vi "Depth count VI.vi"(5 "MS_Total Con and T":cluster{dbl[], dbl[], dbl[], dbl[], i32[]}, 6 "Date":string, 7 "Total Con and T":T1, 8 "error in":errorcluster caption="エラー入力", 9 "Folder Path":string, 10 "Sample Sequence":string, 11 "Cutted Sample Sequence":string) -> (0 "error out":errorcluster caption="エラー出力")   [LabVIEW 2018]
panel:
  out "MS_B Table":string[][](table) caption="B Table"
  out "B Table":string[][](table)
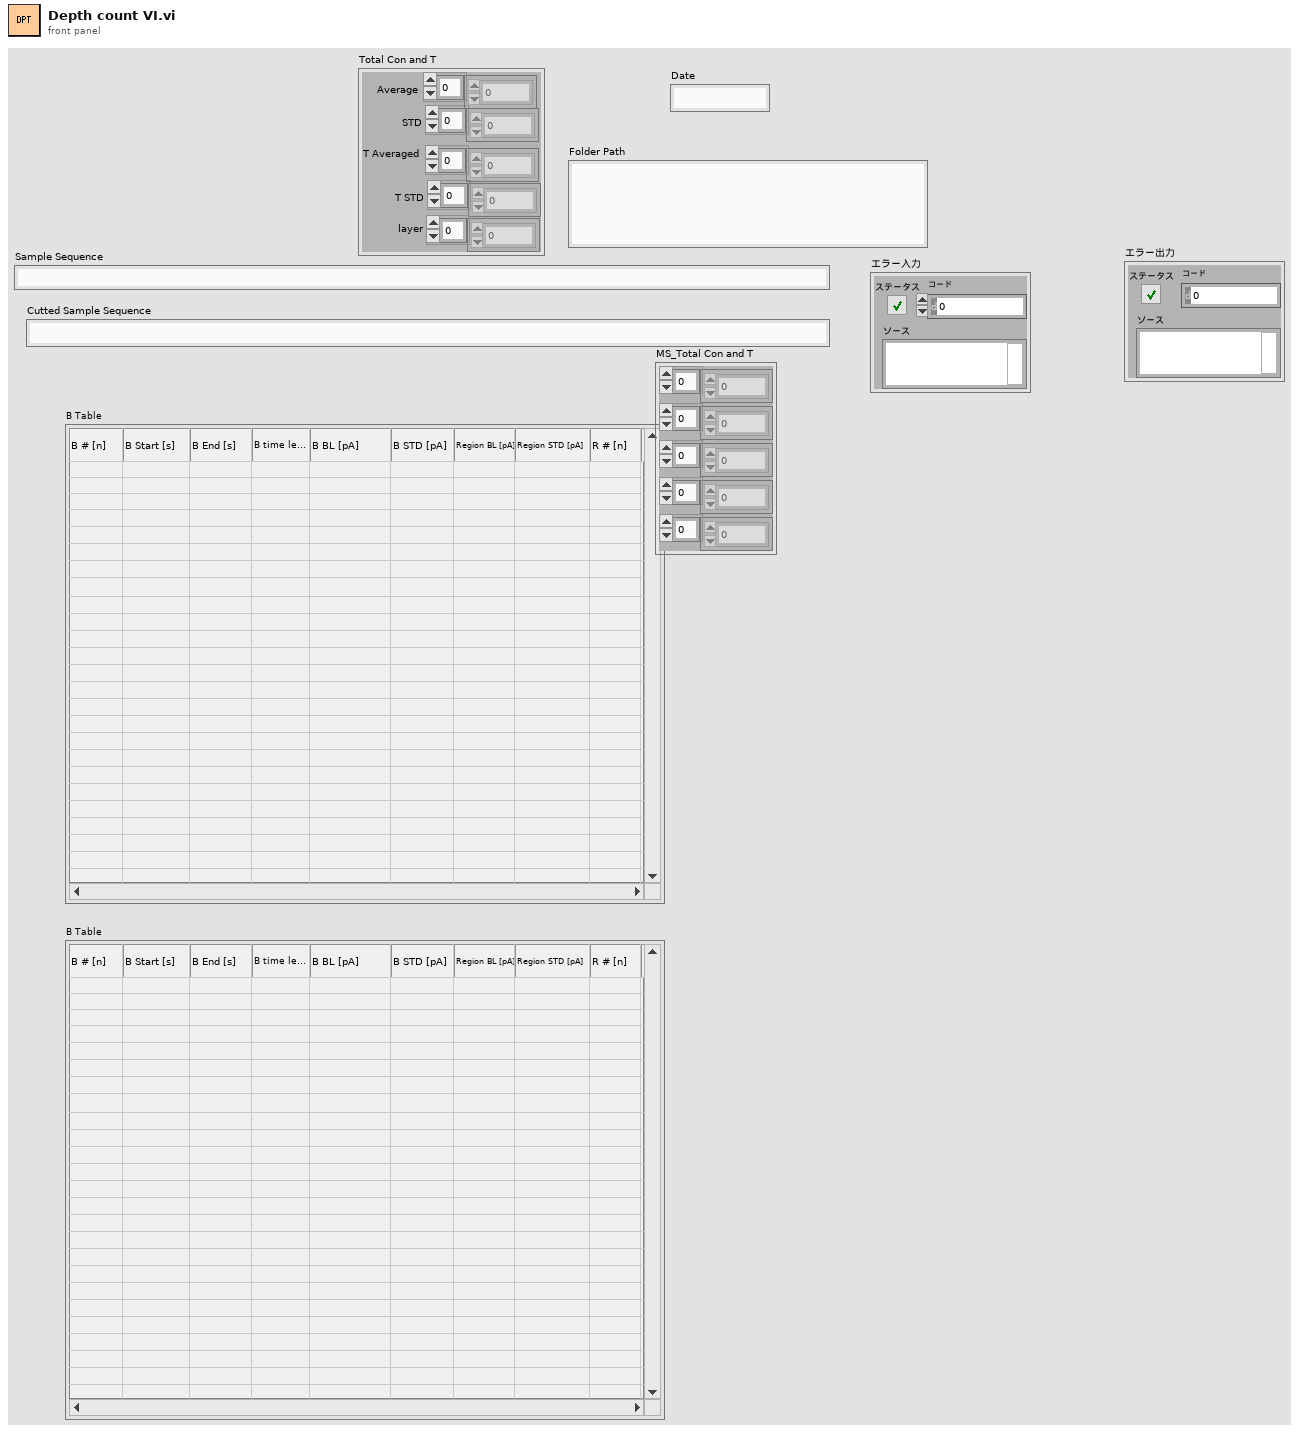
[diagram p1: front panel]
types:
  T1 = cluster{"Average":dbl[], "STD":dbl[], "T Averaged":dbl[], "T STD":dbl[], "layer":i32[]}
  T2 = enum16{"open", "replace", "create", "open or create", "replace or create", "replace or create with confirmation"}
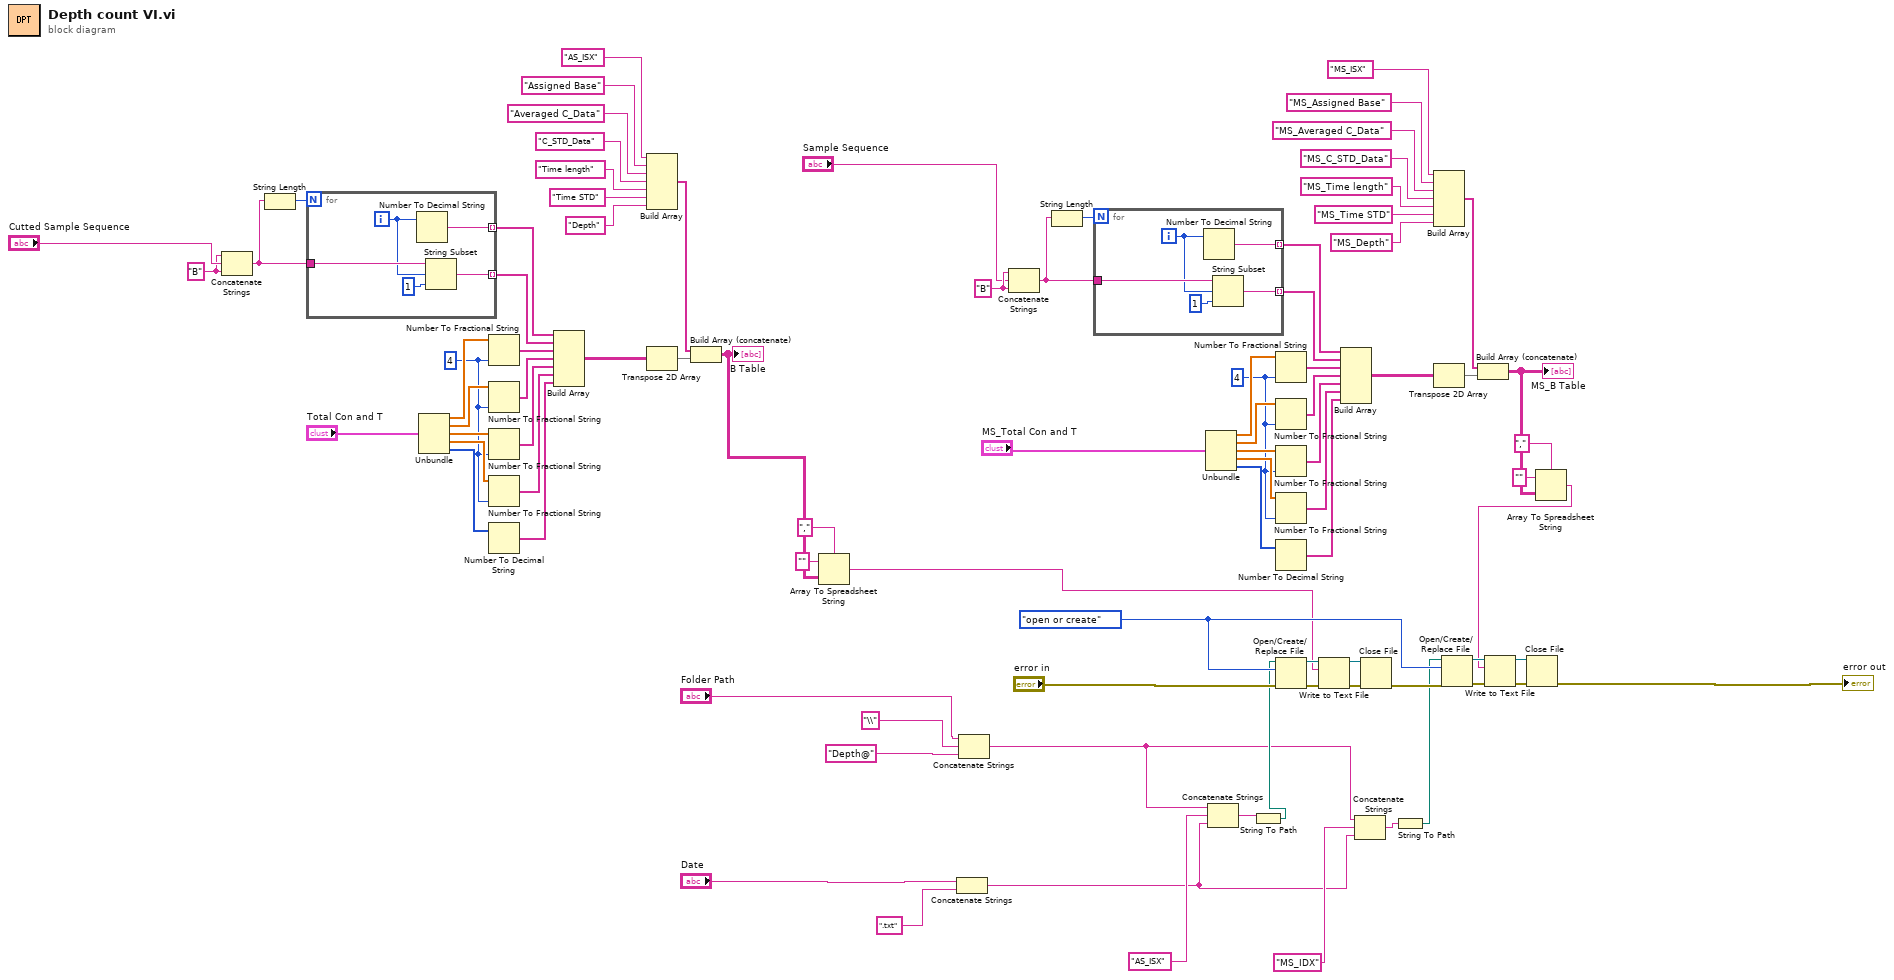
[diagram p0: block diagram]
diagram:
  w21 = T2."open or create" ("操作（0:open）")
  w49 = "B" ("string")
  w56 = i16 4 ("precision (6)")
  w75 = "B" ("string")
  w83 = i16 4 ("precision (6)")
  n1 = Concatenate Strings(w75, "Cutted Sample Sequence", w75) -> (w73:string)
  n2 = String Length(string=w73) -> (length=w74:i32)
  n3 = for {
    N: w74 -> [_]
    tunnel: w73 -> [w93]
    tunnel: [w92] -> w71 mode=indexing
    tunnel: [w90] -> w72 mode=indexing
    i -> [w91]
    n4 = Number To Decimal String(number=w91) -> (decimal integer string=w90:string)  [unwired: 1 in]
    n5 = String Subset(string=w93, offset (0)=w91, length (rest)=1 ("length (rest)")) -> (substring=w92:string)
  }
  n6 = Unbundle("Total Con and T") -> ("Average"=w88:dbl[], "STD"=w87:dbl[], "T Averaged"=w86:dbl[], "T STD"=w85:dbl[], "layer"=w84:i32[])
  n7 = Number To Fractional String(number=w88, precision (6)=w83) -> (F-format string=w82:string[])  [unwired: 2 in]
  n8 = Number To Fractional String(number=w87, precision (6)=w83) -> (F-format string=w81:string[])  [unwired: 2 in]
  n9 = Number To Fractional String(number=w86, precision (6)=w83) -> (F-format string=w80:string[])  [unwired: 2 in]
  n10 = Number To Fractional String(number=w85, precision (6)=w83) -> (F-format string=w79:string[])  [unwired: 2 in]
  n11 = Number To Decimal String(number=w84) -> (decimal integer string=w78:string[])  [unwired: 1 in]
  n12 = Build Array(w72, w71, w82, w81, w80, w79, w78) -> (w77:string[][])
  n13 = Build Array("AS_ISX" ("string"), "Assigned Base" ("string"), "Averaged C_Data" ("string"), "C_STD_Data" ("string"), "Time length" ("string"), "Time STD" ("string"), "Depth" ("string")) -> (w62:string[])
  n14 = Transpose 2D Array(2D array=w77) -> (transposed array=w63:string[][])
  n15 = Build Array (concatenate)(w62, w63) -> (w2:string[][])
  "B Table" <- w2
  n16 = Array To Spreadsheet String(delimiter (Tab)=",", array=w2, 3:"" ("format string")) -> (spreadsheet string=w1:string)
  n17 = Concatenate Strings("Date", ".txt" ("文字列")) -> (w12:string)
  n18 = Concatenate Strings("Folder Path", "\\" ("文字列"), "Depth@" ("文字列")) -> (w11:string)
  n19 = Concatenate Strings(w49, "Sample Sequence", w49) -> (w47:string)
  n20 = String Length(string=w47) -> (length=w48:i32)
  n21 = for {
    N: w48 -> [_]
    tunnel: w47 -> [w98]
    tunnel: [w97] -> w45 mode=indexing
    tunnel: [w95] -> w46 mode=indexing
    i -> [w96]
    n22 = Number To Decimal String(number=w96) -> (decimal integer string=w95:string)  [unwired: 1 in]
    n23 = String Subset(string=w98, offset (0)=w96, length (rest)=1 ("length (rest)")) -> (substring=w97:string)
  }
  n24 = Unbundle("MS_Total Con and T") -> (w61:dbl[], w60:dbl[], w59:dbl[], w58:dbl[], w57:i32[])
  n25 = Concatenate Strings(w11, "AS_ISX" ("文字列"), w12) -> (w16:string)
  n26 = String To Path(string=w16) -> (path=w15:path)
  n27 = Number To Fractional String(number=w61, precision (6)=w56) -> (F-format string=w55:string[])  [unwired: 2 in]
  n28 = Number To Fractional String(number=w60, precision (6)=w56) -> (F-format string=w54:string[])  [unwired: 2 in]
  n29 = Number To Fractional String(number=w59, precision (6)=w56) -> (F-format string=w53:string[])  [unwired: 2 in]
  n30 = Number To Fractional String(number=w58, precision (6)=w56) -> (F-format string=w52:string[])  [unwired: 2 in]
  n31 = Number To Decimal String(number=w57) -> (decimal integer string=w51:string[])  [unwired: 1 in]
  n32 = Open/Create/Replace File(file path (use dialog)=w15, error in="error in", operation (0:open)=w21) -> (refnum out=w30:refnum<file>, error out=w31:errorcluster)  [unwired: 3 in, 1 out]
  n33 = Write to Text File(file (use dialog)=w30, text=w1, error in=w31) -> (refnum out=w29:refnum<file>, error out=w28:errorcluster)  [unwired: 1 in, 1 out]
  n34 = Build Array(w46, w45, w55, w54, w53, w52, w51) -> (w50:string[][])
  n35 = Concatenate Strings(w11, "MS_IDX" ("文字列"), w12) -> (w14:string)
  n36 = Close File(refnum=w29, error in=w28) -> (error out=w22:errorcluster)  [unwired: 1 out]
  n37 = String To Path(string=w14) -> (path=w13:path)
  n38 = Build Array("MS_ISX" ("string"), "MS_Assigned Base" ("string"), "MS_Averaged C_Data" ("string"), "MS_C_STD_Data" ("string"), "MS_Time length" ("string"), "MS_Time STD" ("string"), "MS_Depth" ("string")) -> (w36:string[])
  n39 = Transpose 2D Array(2D array=w50) -> (transposed array=w37:string[][])
  n40 = Open/Create/Replace File(file path (use dialog)=w13, error in=w22, operation (0:open)=w21) -> (refnum out=w26:refnum<file>, error out=w27:errorcluster)  [unwired: 3 in, 1 out]
  n41 = Build Array (concatenate)(w36, w37) -> (w8:string[][])
  "MS_B Table" <- w8
  n42 = Array To Spreadsheet String(delimiter (Tab)=",", array=w8, 3:"" ("format string")) -> (spreadsheet string=w5:string)
  n43 = Write to Text File(file (use dialog)=w26, text=w5, error in=w27) -> (refnum out=w25:refnum<file>, error out=w24:errorcluster)  [unwired: 1 in, 1 out]
  n44 = Close File(refnum=w25, error in=w24) -> (error out=→"error out":errorcluster)  [unwired: 1 out]
